vi "Write Conf File Path.vi"(8 "error in":errorcluster, 10 "Conf File Path":path, 11 "Generic Test Stand in":refnum<class "Generic Test Stand.lvclass">) -> (0 "error out":errorcluster, 3 "Generic Test Stand out":refnum<class "Generic Test Stand.lvclass">)   [LabVIEW 2019, in "Generic Test Stand.lvclass"]
uses:
  Generic Test Stand.lvclass
  Generic Test Stand.lvclass/Generic Test Stand.ctl
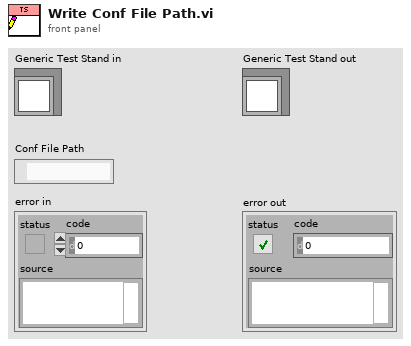
[diagram p1: front panel]
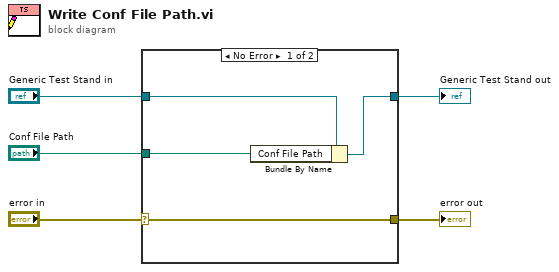
[diagram p0: block diagram]
diagram:
  n1 = case shown="No Error" "error in" {
    selector: "error in" -> [w6 w11]
    tunnel: [w9 w10] -> w4
    tunnel: "Conf File Path" -> [w8 _]
    tunnel: "Generic Test Stand in" -> [w7 w10]
    tunnel: [w6 w11] -> w2
    frame No Error {
      n2 = Bundle By Name(cluster=w7, "Conf File Path"=w8) -> (w9:refnum<class "Generic Test Stand.lvclass">)
    }
    frame Error {
    }
  }
  "Generic Test Stand out" <- w4
  "error out" <- w2
